vi "Create JSON Object.vi"(8 "error in (no error)":errorcluster) -> (0 "error out":errorcluster, 3 "json class out":refnum<class "json class.lvclass">)   [LabVIEW 2021]
uses:
  json class.lvclass
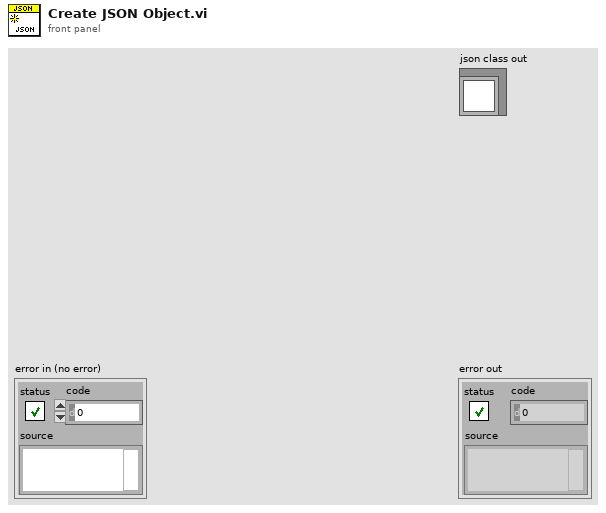
[diagram p1: front panel]
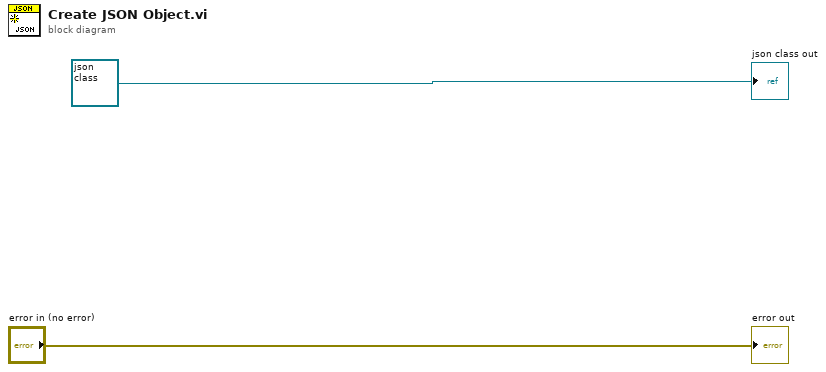
[diagram p0: block diagram]
diagram:
  "error out" <- "error in (no error)"
  "json class out" <- refnum<class "json class.lvclass"> refnum ("json class in")
